vi "Cycle_Finish.vi"(8 "error in (no error)":errorcluster={"status"=FALSE, "code"=0, "source"="\"\""}, 10 "target_cycles":i32=10, 11 "completed_cycles":i32=5) -> (0 "error out":errorcluster={"status"=FALSE, "code"=0, "source"="\"\""}, 3 "all_cycles_done":bool)   [LabVIEW 2026]
doc: "INTENT: Evaluate test endurance cycle count and determine if sequence should loop or finish."
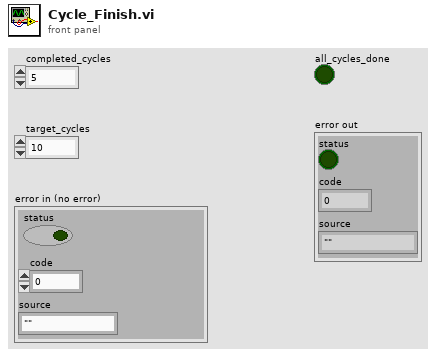
[diagram p1: front panel]
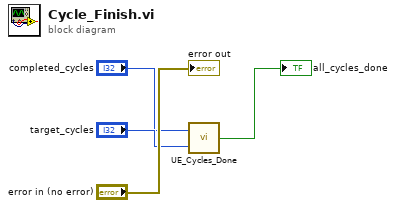
[diagram p0: block diagram]
diagram:
  n1 = call "UE_Cycles_Done.vi"("requested"="target_cycles", "completed"="completed_cycles") -> ("done"=→"all_cycles_done":bool)
  "error out" <- "error in (no error)"
